vi "Read Recorder8400 File.vi"(11 "Path":path=path "D:/同步空间/曲线生成/原始曲线/7、记录仪8400--工作簿1.xlsx") -> (3 "Data Series":T1[](array[typedef]))   [LabVIEW 2020, in "Data Viewer.lvlib"]
uses:
  Data Viewer.lvlib
  Data Serie--cluster.ctl
  File Type--enum.ctl
  <vilib>/Utility/file.llb/Read Delimited Spreadsheet (string).vi
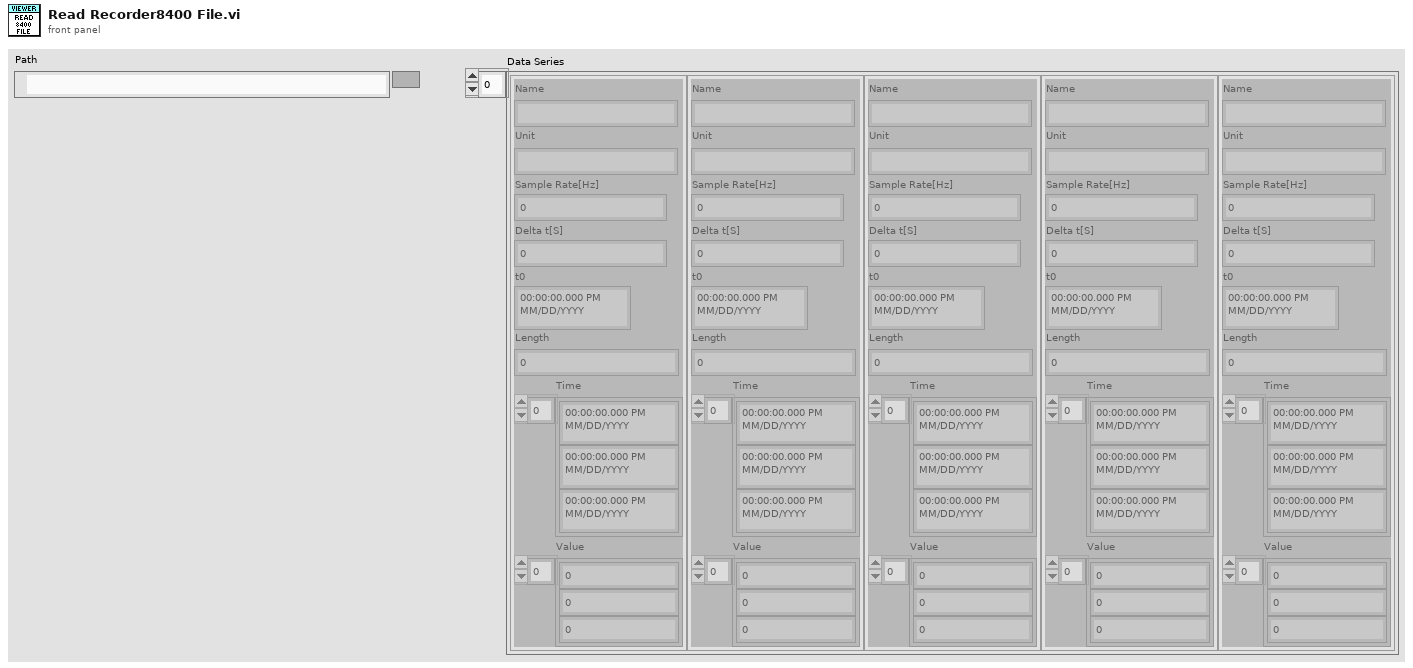
[diagram p1: front panel]
types:
  T1 = typedef "Data Viewer.lvlib/Data Serie--cluster.ctl" = cluster{"Name":string, "Unit":string, "Sample Rate[Hz]":dbl, "Delta t[S]":dbl, "t0":timestamp, "Length":i32, "Time":timestamp[], "Value":dbl[]}
  T2 = typedef "Data Viewer.lvlib/File Type--enum.ctl" = enum16{"伟思环境箱", "增达环境箱", "广五所环境箱", "无纸记录仪", "帕捷SA00339", "记录仪840", "记录仪8400", "记录仪MR888", "*.csv"}
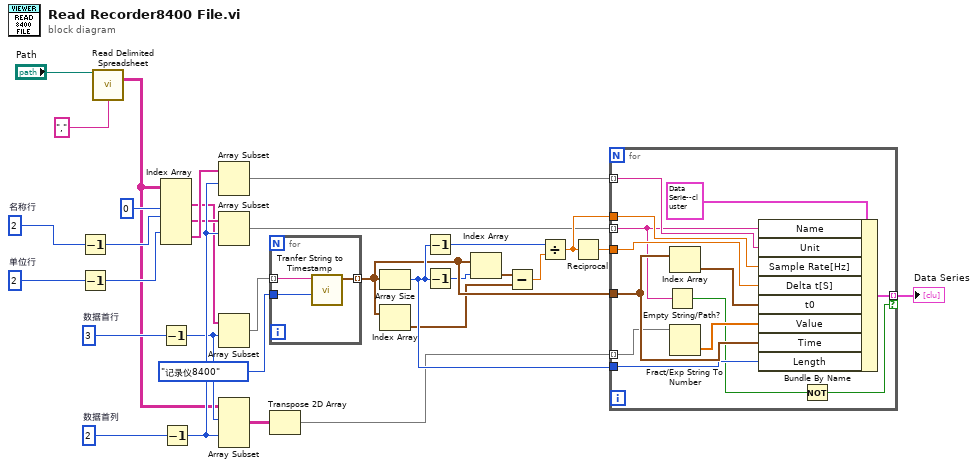
[diagram p0: block diagram]
diagram:
  w11 = 2  # 数据首列
  w10 = 3  # 数据首行
  w8 = 2  # 单位行
  w6 = 2  # 名称行
  n1 = Decrement(x=w6) -> (x-1=w15:i32)
  n2 = Decrement(x=w8) -> (x-1=w16:i32)
  n3 = call-poly <vilib>:"Read Delimited Spreadsheet.vi"("file path (dialog if empty)"="Path", "delimiter (\\t)"="," ("delimiter (\\t)")) -> ("all rows"=w2:string[][])  [unwired: 8 in, 5 out]
  n4 = Index Array(array=w2, index (col) #1=0 ("disabled index (col)"), index (row) #2=w15, index (row) #3=w16) -> (element #1=w5:string[], element #2=w7:string[], element #3=w9:string[])  [unwired: 3 in]
  n5 = Decrement(x=w10) -> (x-1=w17:i32)
  n6 = Decrement(x=w11) -> (x-1=w18:i32)
  n7 = Array Subset(array=w9, index=w18) -> (w14:string[])  [unwired: 1 in]
  n8 = Array Subset(array=w7, index=w18) -> (w13:string[])  [unwired: 1 in]
  n9 = Array Subset(array=w5, index=w17) -> (w27:string[])  [unwired: 1 in]
  n10 = Array Subset(array=w2, index (row)=w17, index (col)=w18) -> (w12:string[][])  [unwired: 2 in]
  n11 = for {
    tunnel: [w34] -> w28 mode=indexing
    tunnel: w27 -> [w33] mode=indexing
    tunnel: File_Type--enum."记录仪8400" ("File Type") -> [w32]
    n12 = call "Tranfer String to Timestamp.vi"("File Type"=w32, "String"=w33) -> ("time stamp"=w34:timestamp)  [unwired: 9 in]
  }
  n13 = Transpose 2D Array(2D array=w12) -> (transposed array=w19:string[][])
  n14 = Array Size(array=w28) -> (size(s)=w31:i32)
  n15 = Index Array(array=w28) -> (element=w22:timestamp)  [unwired: 1 in]
  n16 = Decrement(x=w31) -> (x-1=w30:i32)
  n17 = Decrement(x=w31) -> (x-1=w20:i32)
  n18 = Index Array(array=w28, index=w20) -> (element=w21:timestamp)
  n19 = Subtract(x=w21, y=w22) -> (x-y=w23:dbl)
  n20 = Divide(x=w30, y=w23) -> (x/y=w24:dbl)
  n21 = Reciprocal(x=w24) -> (1/x=w25:dbl)
  n22 = for {
    tunnel: w13 -> [w35] mode=indexing
    tunnel: w14 -> [w39] mode=indexing
    tunnel: w19 -> [w44] mode=indexing
    tunnel: w28 -> [w45]
    tunnel: w24 -> [w42]
    tunnel: w25 -> [w41]
    tunnel: [w40] -> w26 mode=indexing if=w36
    tunnel: w31 -> [w38]
    n23 = Empty String/Path?(string/path=w35) -> (empty?=w37:bool)
    n24 = Index Array(array=w45) -> (element=w46:timestamp)  [unwired: 1 in]
    n25 = Fract/Exp String To Number(string=w44) -> (number=w43:dbl[])  [unwired: 3 in, 1 out]
    n26 = Bundle By Name(cluster=T1 {"Name"="", "Unit"="", "Sample Rate[Hz]"=0.0, "Delta t[S]"=0.0, "t0"=timestamp(0 s since 1904-01-01), "Length"=0, "Time"=[], "Value"=[]} ("Data Serie"), "Name"=w35, "Unit"=w39, "Sample Rate[Hz]"=w42, "Delta t[S]"=w41, "t0"=w46, "Value"=w43, "Time"=w45, "Length"=w38) -> (w40:T1)
    n27 = Not(x=w37) -> (.not. x?=w36:bool)
  }
  "Data Series" <- w26
